vi "constant-command.vi"(11 "error in":errorcluster) -> (15 "error out":errorcluster)   [LabVIEW 2024]
doc: "Static analysis fixture. Do not run."
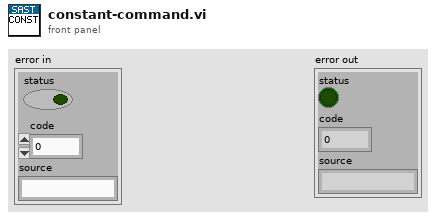
[diagram p1: front panel]
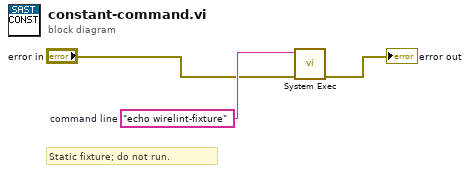
[diagram p0: block diagram]
diagram:
  w2 = "echo wirelint-fixture"  # command line
  # "Static fixture; do not run."
  n1 = call <vilib>:"System Exec.vi"("error in (no error)"="error in", "command line"=w2) -> ("error out"=→"error out":errorcluster)  [unwired: 6 in, 3 out]
